vi "Test_One_Point_Sim.vi"(8 "error in (no error)":errorcluster={"status"=FALSE, "code"=0, "source"="\"\""}, 10 "Target Pressure (bar)":dbl=100.0, 11 "Start (True to run)":bool=TRUE) -> (0 "error out":errorcluster={"status"=FALSE, "code"=0, "source"="\"\""}, 1 "Simulated Time (ms)":i64, 2 "Test Passed":bool, 3 "Harness Result":string)   [LabVIEW 2026]
doc: "INTENT: Unit test harness executing first working slice (one configurable operating point in simulation) as specified in docs/labview/09_FIRST_WORKING_SLICE.md."
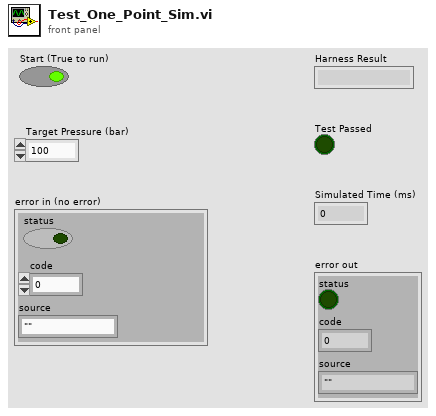
[diagram p1: front panel]
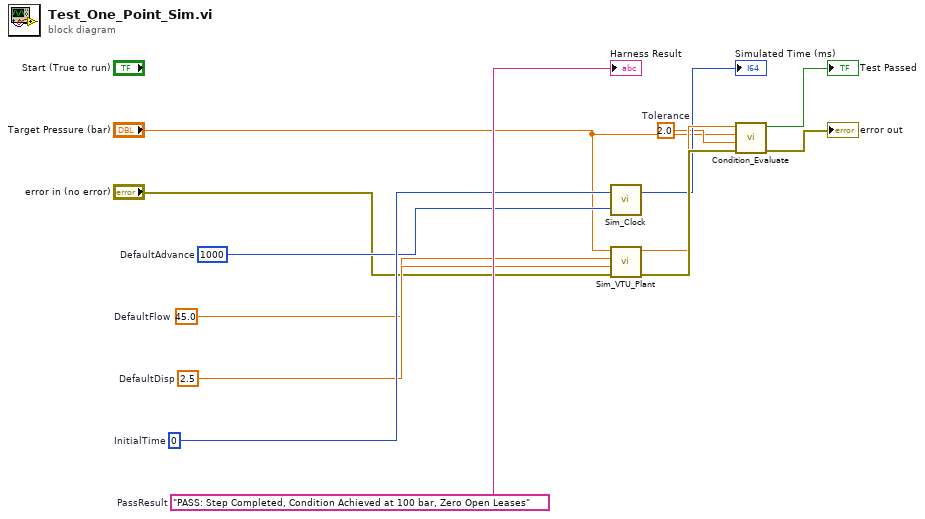
[diagram p0: block diagram]
diagram:
  w13 = "PASS: Step Completed, Condition Achieved at 100 bar, Zero Open Leases"  # PassResult
  w7 = i64 0  # InitialTime
  w6 = 2.0  # Tolerance
  w5 = 2.5  # DefaultDisp
  w4 = 45.0  # DefaultFlow
  w3 = i64 1000  # DefaultAdvance
  n1 = call "Sim_Clock.vi"("advance_ms"=w3, "current_ms"=w7) -> ("next_ms"=→"Simulated Time (ms)":i64)  [unwired: 1 out]
  n2 = call "Sim_VTU_Plant.vi"("error in (no error)"="error in (no error)", "displacement_sp"=w5, "flow_sp"=w4, "pressure_sp"="Target Pressure (bar)") -> ("error out"=w10:errorcluster, "act_pressure"=w9:dbl)  [unwired: 4 in, 2 out]
  n3 = call "Condition_Evaluate.vi"("error in (no error)"=w10, "tolerance"=w6, "target_setpoint"="Target Pressure (bar)", "actual_value"=w9) -> ("error out"=→"error out":errorcluster, "condition_met"=→"Test Passed":bool)  [unwired: 6 in]
  "Harness Result" <- w13
